vi "Generate Failure Nodes.vi"(8 "error in (no error)":errorcluster, 10 "Result":T1, 11 "XML Report in":refnum<class "XML Report.lvclass">) -> (0 "error out":errorcluster, 3 "XML Report out":refnum<class "XML Report.lvclass">)   [LabVIEW 2020, in "XML Report.lvclass"]
uses:
  XML Report.lvclass
  Core/Result/Result.ctl
  Core/Result/Status.ctl
  Core/Result/Type.ctl
  XML Report.lvclass/XML Report.ctl
  <vilib>/Utility/miscctls.llb/LVMapReplaceAction.ctl
  <resource>/objmgr/DOMUserDefRef.rc
  Framework/Utilities/Utilities.lvlib
  Core/Result/Result.lvlib
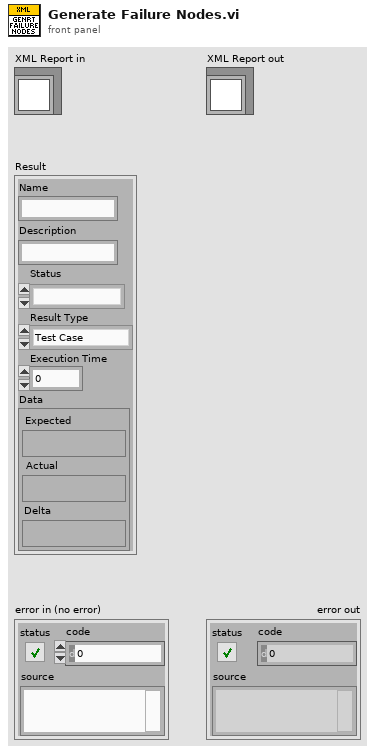
[diagram p1: front panel]
types:
  T1 = typedef "Result.lvlib/Result.ctl" = cluster{"Name":string, "Description":string, "Status":T2, "Result Type":T3, "Execution Time":dbl, "Data":cluster{"Expected":variant, "Actual":variant, "Delta":variant}}
  T2 = typedef "Result.lvlib/Status.ctl" = enum16{"", "Passed", "Failed", "Error", "Skipped", "Setup Error", "Broken", "Teardown Error"}
  T3 = typedef "Result.lvlib/Type.ctl" = enum16{"Test Case", "Test Suite", "Test Run", "Pass", "Fail", "Skip", "Pass if", "Fail if", "Pass if Error", "Fail if Error", "Pass if Equal", "Fail if Equal"}
  T4 = typedef "LVMapReplaceAction.ctl" = enum32{"Modify Entry only if found", "Add or Modify Entry", "Delete Entry"}
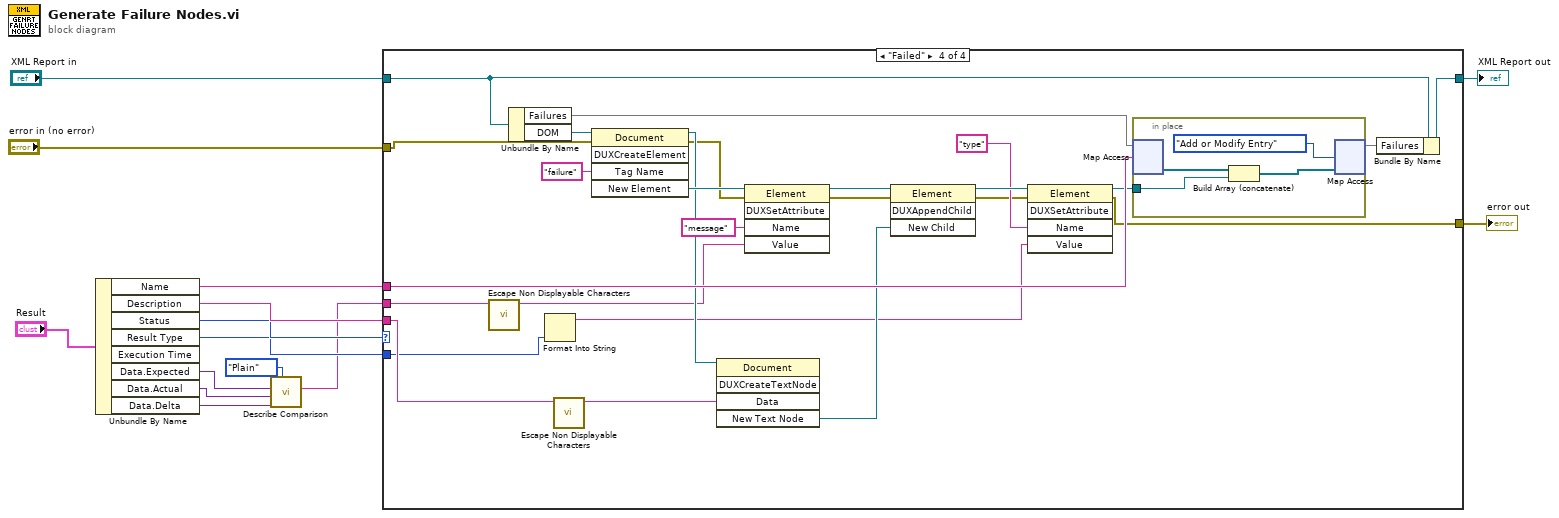
[diagram p0: block diagram]
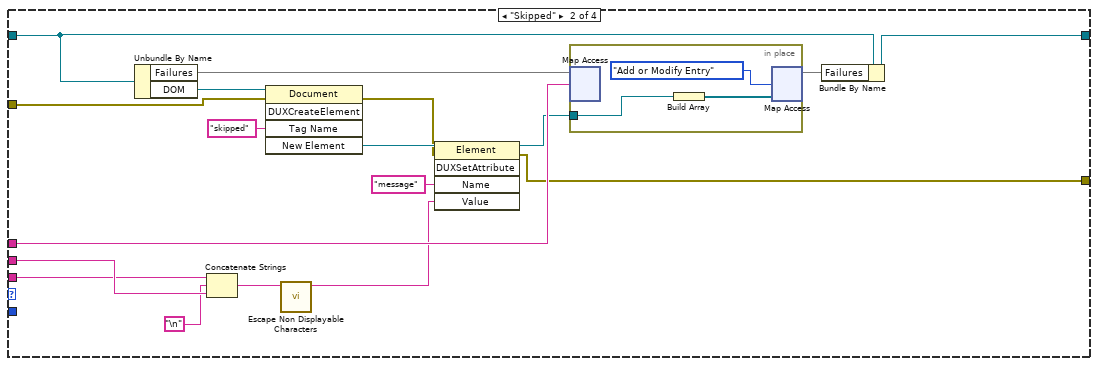
[diagram p3: hidden frame]
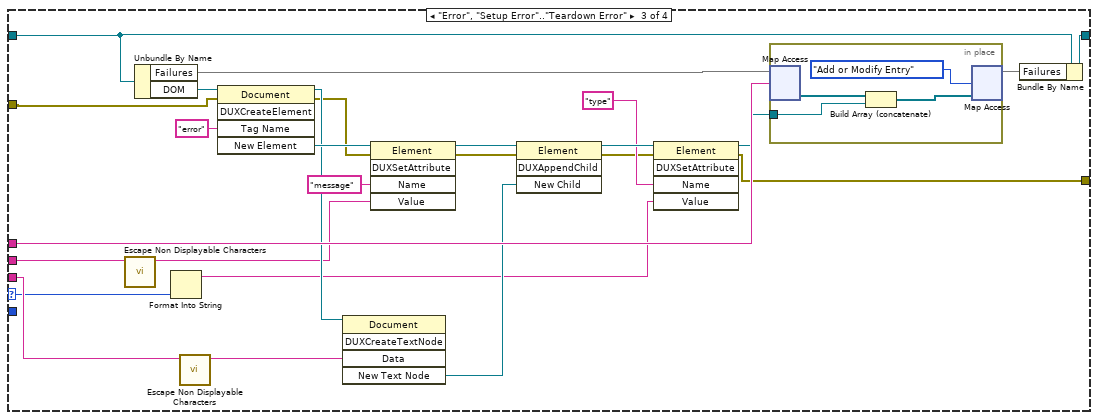
[diagram p4: hidden frame]
diagram:
  n1 = Unbundle By Name("Result") -> ("Name"=w11:string, "Description"=w10:string, "Status"=w9:T2, "Result Type"=w8:T3, "Data.Expected"=w7:variant, "Data.Actual"=w6:variant, "Data.Delta"=w5:variant)  [unwired: 1 out]
  n2 = call "Describe Comparison.vi"("Delta"=w5, "Style"=enum16{"Diff", "Plain"}."Plain", "Actual"=w6, "Expected"=w7) -> ("Description"=w4:string)  [unwired: 7 in]
  n3 = case shown="\"Failed\"" w9 {
    selector: w9 -> [_ _ w45 _]
    tunnel: [w16 w34 w63 w93] -> w13
    tunnel: "XML Report in" -> [w16 w33 w62 w92]
    tunnel: w11 -> [_ w29 w58 w88]
    tunnel: w4 -> [_ w24 w42 w84]
    tunnel: w10 -> [_ w22 w53 w82]
    tunnel: w8 -> [_ _ _ w73]
    tunnel: "error in (no error)" -> [w15 w19 w40 w70]
    tunnel: [w15 w17 w39 w68] -> w1
    frame "", "Passed" {
    }
    frame "Skipped" {
      n4 = Unbundle By Name(w33) -> ("Failures"=w30:map{string, refnum<k20>[]}, "DOM"=w32:refnum<k20>)
      n5 = Concatenate Strings(w22, "\n", w24) -> (w23:string)
      n6 = invoke class="Document" method="DUXCreateElement"(reference=w32, error in=w19, "Tag Name"="skipped") -> (error out=w18:errorcluster, "New Element"=w28:refnum<k20>)  [unwired: 2 in, 3 out]
      n7 = call "Escape Non Displayable Characters.vi"("Raw String"=w23) -> ("Escaped String"=w20:string)  [unwired: 10 in]
      n8 = invoke class="Element" method="DUXSetAttribute"(reference=w28, error in=w18, "Name"="message", "Value"=w20) -> (reference out=w26:refnum<k20>, error out=w17:errorcluster)  [unwired: 1 in, 3 out]
      n9 = in-place {
        in-place-border: w26 -> [w37]
        n10 = in-place-map #1(w30, w29) -> ()  [unwired: 1 in, 2 out]
        n11 = Build Array(w37) -> (w35:refnum<k20>[])
        n12 = in-place-map #1(w35, LVMapReplaceAction."Add or Modify Entry" ("action")) -> (w27:map{string, refnum<k20>[]})  [unwired: 2 out]
      }
      n13 = Bundle By Name(cluster=w33, "Failures"=w27) -> (w34:refnum<class "XML Report.lvclass">)
    }
    frame "Error", "Setup Error".."Teardown Error" {
      n14 = call "Escape Non Displayable Characters.vi"("Raw String"=w42) -> ("Escaped String"=w41:string)  [unwired: 10 in]
      n15 = Unbundle By Name(w62) -> ("Failures"=w59:map{string, refnum<k20>[]}, "DOM"=w61:refnum<k20>)
      n16 = Format Into String(w45) -> (resulting string=w44:string)  [unwired: 3 in, 1 out]
      n17 = call "Escape Non Displayable Characters.vi"("Raw String"=w53) -> ("Escaped String"=w43:string)  [unwired: 10 in]
      n18 = invoke class="Document" method="DUXCreateElement"(reference=w61, error in=w40, "Tag Name"="error") -> (reference out=w54:refnum<k20>, error out=w49:errorcluster, "New Element"=w57:refnum<k20>)  [unwired: 2 in, 2 out]
      n19 = invoke class="Document" method="DUXCreateTextNode"(reference=w54, "Data"=w43) -> ("New Text Node"=w50:refnum<k20>)  [unwired: 3 in, 4 out]
      n20 = invoke class="Element" method="DUXSetAttribute"(reference=w57, error in=w49, "Name"="message", "Value"=w41) -> (reference out=w52:refnum<k20>, error out=w48:errorcluster)  [unwired: 1 in, 3 out]
      n21 = invoke class="Element" method="DUXAppendChild"(reference=w52, error in=w48, "New Child"=w50) -> (reference out=w51:refnum<k20>, error out=w38:errorcluster)  [unwired: 1 in, 2 out]
      n22 = invoke class="Element" method="DUXSetAttribute"(reference=w51, error in=w38, "Name"="type", "Value"=w44) -> (reference out=w47:refnum<k20>, error out=w39:errorcluster)  [unwired: 1 in, 3 out]
      n23 = in-place {
        in-place-border: w47 -> [w66]
        n24 = in-place-map #2(w59, w58) -> (w67:refnum<k20>[])  [unwired: 1 in, 1 out]
        n25 = Build Array (concatenate)(w67, w66) -> (w64:refnum<k20>[])
        n26 = in-place-map #2(w64, LVMapReplaceAction."Add or Modify Entry" ("action")) -> (w56:map{string, refnum<k20>[]})  [unwired: 2 out]
      }
      n27 = Bundle By Name(cluster=w62, "Failures"=w56) -> (w63:refnum<class "XML Report.lvclass">)
    }
    frame "Failed" {
      n28 = call "Escape Non Displayable Characters.vi"("Raw String"=w84) -> ("Escaped String"=w72:string)  [unwired: 10 in]
      n29 = Unbundle By Name(w92) -> ("Failures"=w89:map{string, refnum<k20>[]}, "DOM"=w91:refnum<k20>)
      n30 = Format Into String(w73) -> (resulting string=w74:string)  [unwired: 3 in, 1 out]
      n31 = call "Escape Non Displayable Characters.vi"("Raw String"=w82) -> ("Escaped String"=w71:string)  [unwired: 10 in]
      n32 = invoke class="Document" method="DUXCreateElement"(reference=w91, error in=w70, "Tag Name"="failure") -> (reference out=w83:refnum<k20>, error out=w78:errorcluster, "New Element"=w87:refnum<k20>)  [unwired: 2 in, 2 out]
      n33 = invoke class="Document" method="DUXCreateTextNode"(reference=w83, "Data"=w71) -> ("New Text Node"=w79:refnum<k20>)  [unwired: 3 in, 4 out]
      n34 = invoke class="Element" method="DUXSetAttribute"(reference=w87, error in=w78, "Name"="message", "Value"=w72) -> (reference out=w81:refnum<k20>, error out=w77:errorcluster)  [unwired: 1 in, 3 out]
      n35 = invoke class="Element" method="DUXAppendChild"(reference=w81, error in=w77, "New Child"=w79) -> (reference out=w80:refnum<k20>, error out=w69:errorcluster)  [unwired: 1 in, 2 out]
      n36 = invoke class="Element" method="DUXSetAttribute"(reference=w80, error in=w69, "Name"="type", "Value"=w74) -> (reference out=w76:refnum<k20>, error out=w68:errorcluster)  [unwired: 1 in, 3 out]
      n37 = in-place {
        in-place-border: w76 -> [w96]
        n38 = in-place-map #3(w89, w88) -> (w97:refnum<k20>[])  [unwired: 1 in, 1 out]
        n39 = Build Array (concatenate)(w97, w96) -> (w94:refnum<k20>[])
        n40 = in-place-map #3(w94, LVMapReplaceAction."Add or Modify Entry" ("action")) -> (w86:map{string, refnum<k20>[]})  [unwired: 2 out]
      }
      n41 = Bundle By Name(cluster=w92, "Failures"=w86) -> (w93:refnum<class "XML Report.lvclass">)
    }
  }
  "XML Report out" <- w13
  "error out" <- w1
